vi "GET Concatenated Control.vi"(0 "url suffix":string, 11 "error in":errorcluster) -> (15 "error out":errorcluster)   [LabVIEW 2024]
doc: "Static analysis fixture with a concatenated control URL and a permanent false guard."
uses:
  <vilib>/httpClient/LabVIEWHTTPClient.lvlib
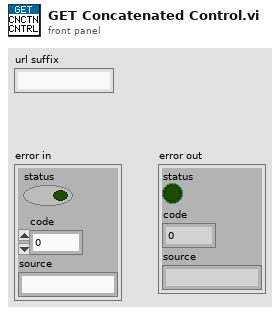
[diagram p1: front panel]
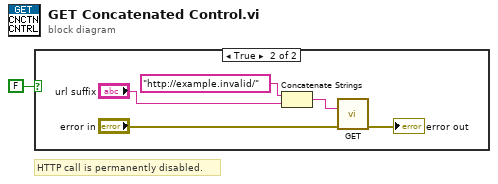
[diagram p0: block diagram]
diagram:
  # "HTTP call is permanently disabled."
  n1 = case shown="True" FALSE ("guard") {
    frame False {
    }
    frame True {
      n2 = Concatenate Strings("http://example.invalid/" ("url prefix"), "url suffix") -> (w5:string)
      n3 = call <vilib>:"GET.vi"("url"=w5, "error in (no error)"="error in") -> ("error out"=→"error out":errorcluster)  [unwired: 10 in, 3 out]
    }
  }
